vi "getOutputOffset.vi"(8 "error in (no error)":errorcluster, 11 "Instrument.Lockin in":refnum<class "Instrument.Lockin.lvclass">) -> (0 "error out":errorcluster, 2 "OutputOffset":dbl[](array[numeric]), 3 "Instrument.Lockin out":refnum<class "Instrument.Lockin.lvclass">)   [LabVIEW 2019, in "Instrument.Lockin.lvlib" / "Instrument.Lockin.lvclass"]
doc: "API to get the output gain on the AO channels.\n\nIf address=\"\", this API reads from localhost\nIf address is remote lockin, you need to add this computer to allowed whitelist on the lockin computer you are trying to access."
uses:
  Instrument.Lockin.lvclass
  Lockin.Typedefs/API/Lockin.Commands--Enum.ctl
  3fbe3561-5f32-4bfe-8563-ec8b7302d399.vi
  <vilib>/PRIrvin/JSON-RPC/API/JSON to Variant.vi
  <vilib>/Utility/Data Type/Get Type Information.vi
  <vilib>/JDP Science/JSONtext/JSON type.vi
  <vilib>/JDP Science/JSONtext/Get Array Elements.vi
  <vilib>/JDP Science/JSONtext/JSON text to Variant.vi
  Lockin.Typedefs/Lockin.Typedefs.lvlib
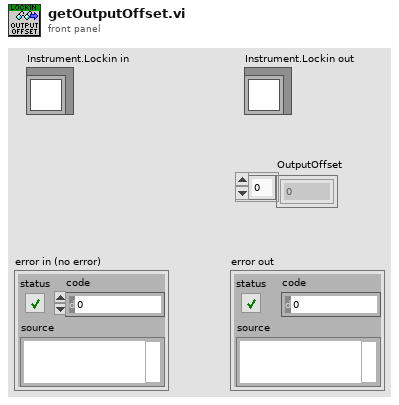
[diagram p1: front panel]
types:
  T1 = typedef "Lockin.Typedefs.lvlib/Lockin.Commands--Enum.ctl" = enum16{"setAO", "setAO_Amplitude", "setAO_DC", "setAO_Frequency", "setAO_Phase", "setAO_Function", "setREF", "setREF_Frequency", "setREF_Phase", "setREF_TC", "setREF_Roll-Off", "setDAQ", "setSampling", "setState", "getState", "getAO", "getAI", "getResults", "getSampling", "getAOconfig", "getREFconfig", "setInputGain", "setOutputGain", "getInputGain", "getOutputGain", "setSweep", "setSweepTime", "setSweepTable", "getStatus", "getSweepResults", "getSweepWaveforms", "logConfiguration", "startLogging", "stopLogging", "setInputOffset", "getInputOffset", "setOutputOffset", "getOutputOffset", "getInputDAQ", "getOutputDAQ", "getLinkFrequency", "setLinkFrequency", "measureInputOffset", "getDevices"}
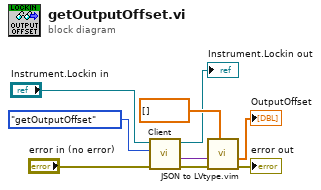
[diagram p0: block diagram]
diagram:
  n1 = call-dynamic "Client.vi"("error in (no error)"="error in (no error)", "Command in"=Lockin.Commands--Enum."getOutputOffset" ("Commands"), "Instrument in"="Instrument.Lockin in") -> ("error out"=w9:errorcluster, "Data out"=w8:variant, "Instrument out"=→"Instrument.Lockin out":refnum<class "Instrument.Lockin.lvclass">)  [unwired: 5 in, 1 out]
  n2 = call "JSON to LVtype.vim"("type"=dbl[] [] ("InputOffset"), "error in (no error)"=w9, "JSON Data in"=w8) -> ("error out"=→"error out":errorcluster, "Data out"=→"OutputOffset":dbl[])  [unwired: 7 in]
